vi "Lab 5.vi"() -> ()   [LabVIEW 2025]
uses:
  Control ENUM.ctl
  Lab 3/Control og.ctl
  Lab 3/Control Runners.ctl
  Lab 3/Control Raw.ctl
  <vilib>/Analysis/baseanly.llb/Mean (DBL).vi
  <vilib>/Instr/_visa.llb/VISA Configure Serial Port (Instr).vi
  <vilib>/Analysis/NI_AALBase.lvlib
panel:
  in  "Enter your name":string
  in  "Play":bool
  in  "Button":bool
  out "Waveform Chart":i32(graph)
  out "XY Graph 2":cluster{i32[], i32[]}(graph)
  out "return count":u32
  out "error out 2":errorcluster
  in  "stop":bool
  out "read buffer":string
  out "Cursor BPM":dbl
  in  "Training Data":path
  out "HEART RATE ZONES":string[][](array[string])
  out "BPM":cluster{"Time":timestamp[], "Bpm":i32[]}(graph)
  out "XY Graph":T1(graph)
  in  "Stop":bool
  in  "Save":bool
  in  "New":bool
  out "error out":errorcluster
  in  "error in":errorcluster
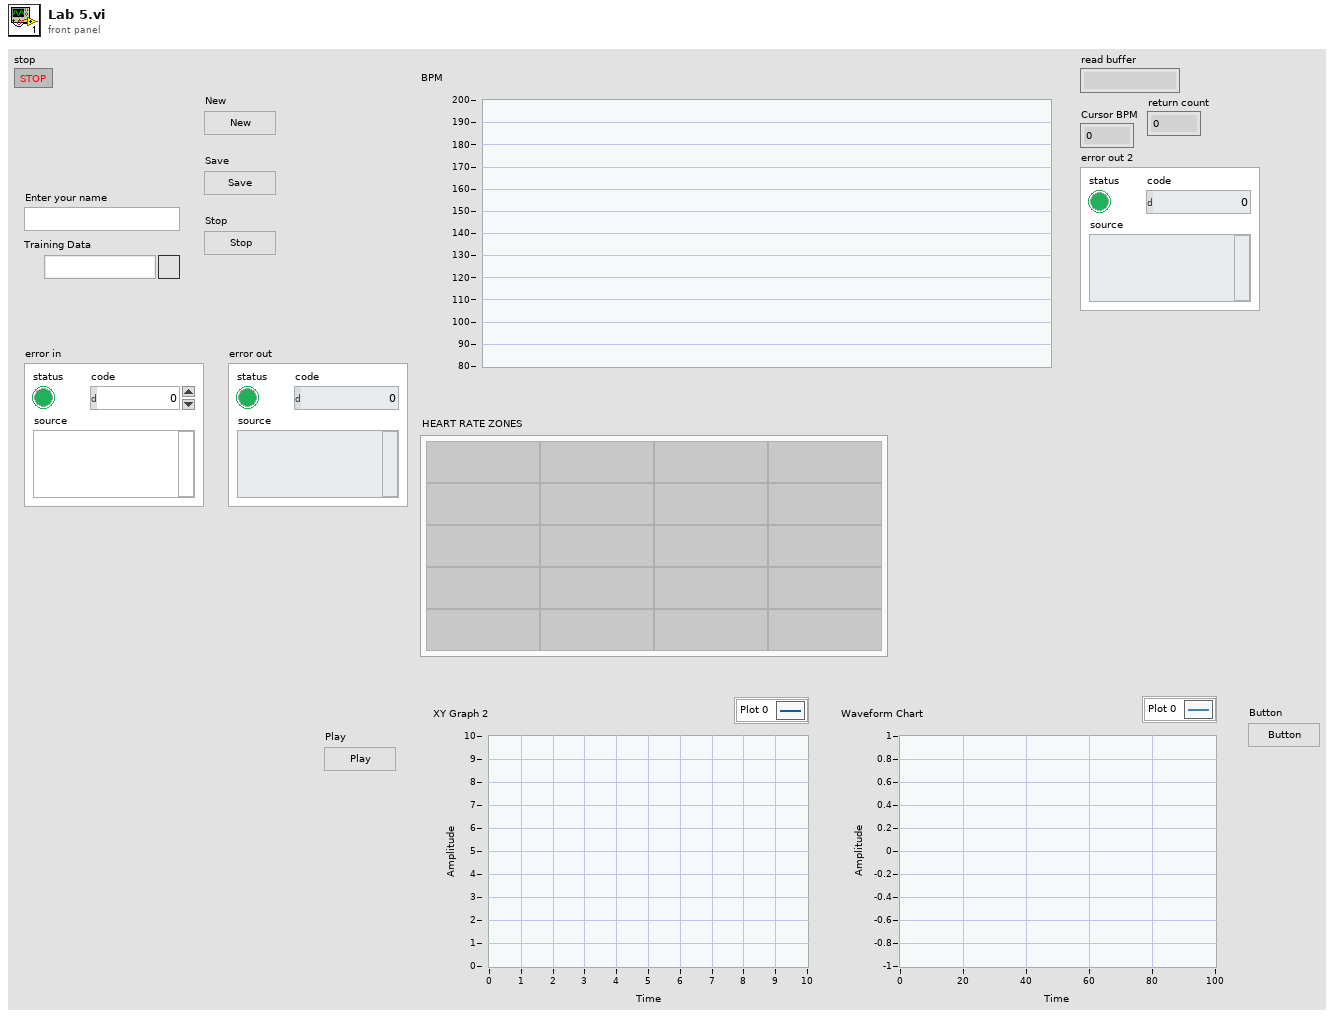
[diagram p1: front panel]
types:
  T1 = cluster{"Total Time in Zone":dbl[], "Heart Rate Zone No":dbl[]}
  T2 = typedef "Control og.ctl" = cluster{"Runner's Data":T3, "HR Max":i32, "Raw Data":T4, "% HR MAX ":dbl[], "HR Zones":string[][], "Heart Rate Zone No":dbl[], "Total Time in Zone":dbl[]}
  T3 = typedef "Control Runners.ctl" = cluster{"Name":string, "Age":i32}
  T4 = typedef "Control Raw.ctl" = cluster{"Time":timestamp[], "Bpm":i32[]}
  T5 = typedef "Control ENUM.ctl" = enum16{"Application Error", "Init", "Idle", "Analyse New Training", "Save", "Error Handling", "Stop", "Play\n"}
  T6 = enum16{"open", "replace", "create", "open or create", "replace or create", "replace or create with confirmation"}
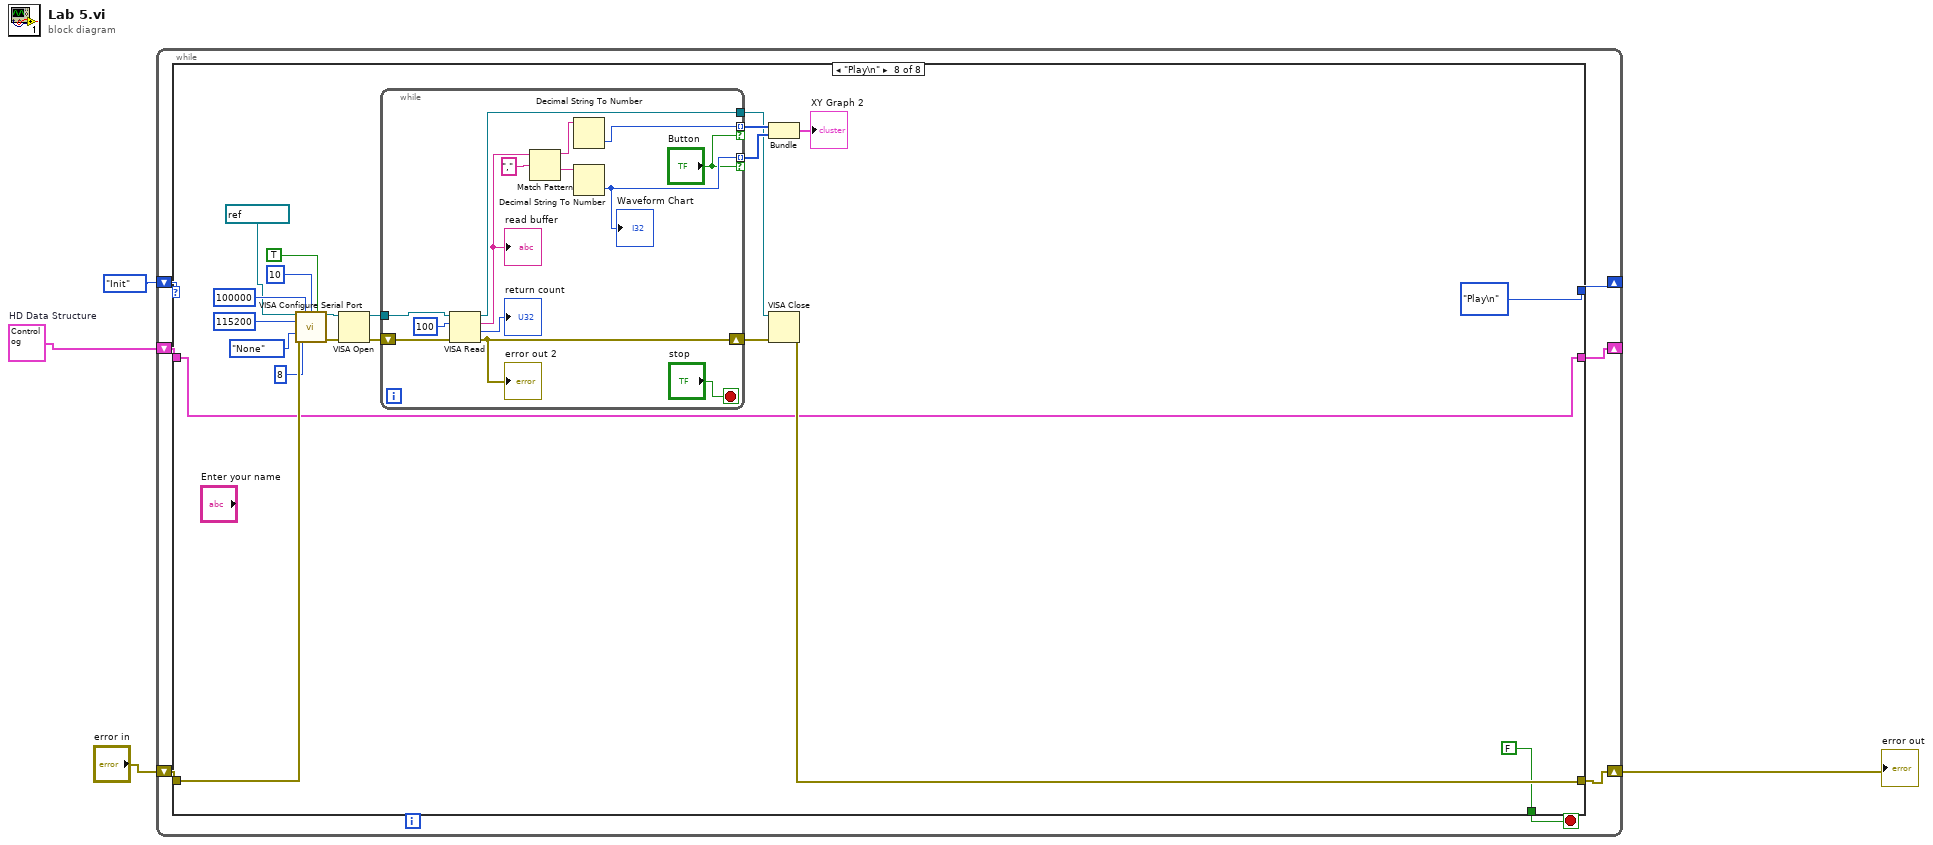
[diagram p0: block diagram]
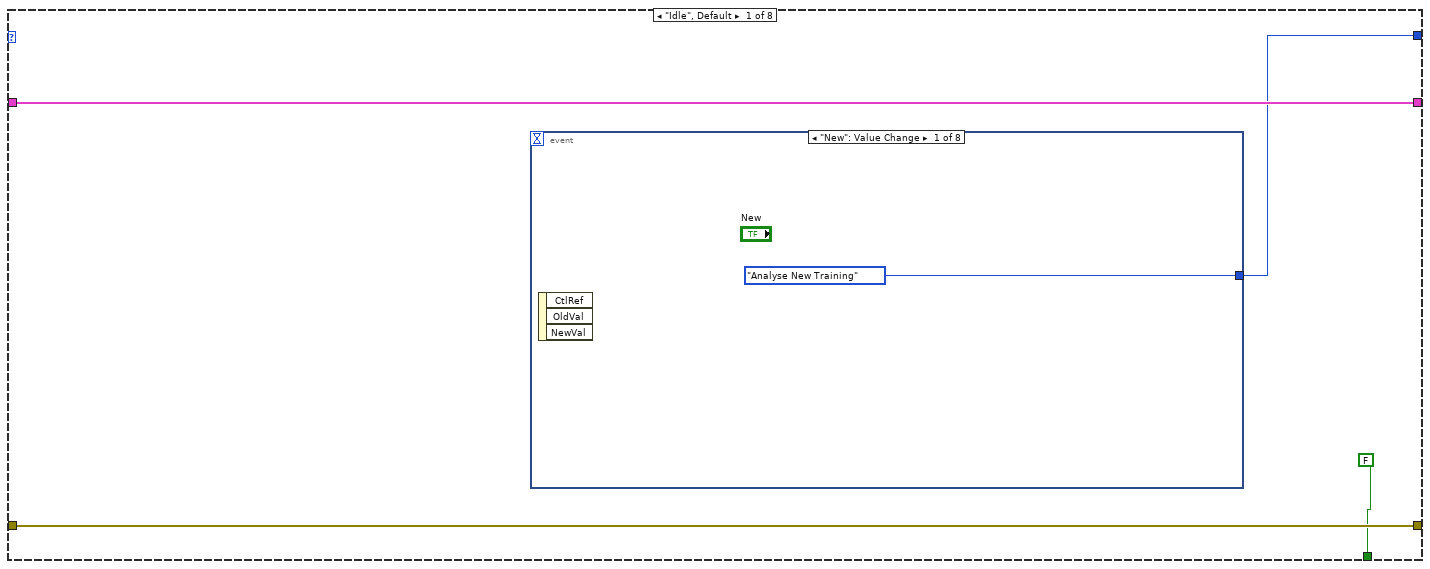
[diagram p2: hidden frame]
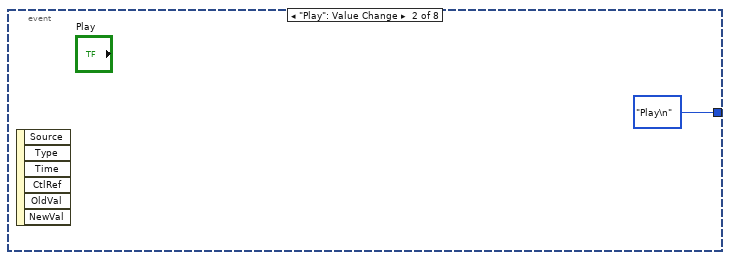
[diagram p3: hidden frame]
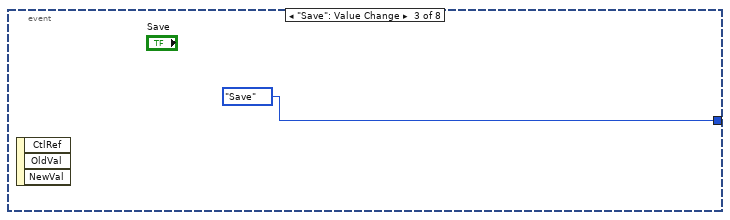
[diagram p4: hidden frame]
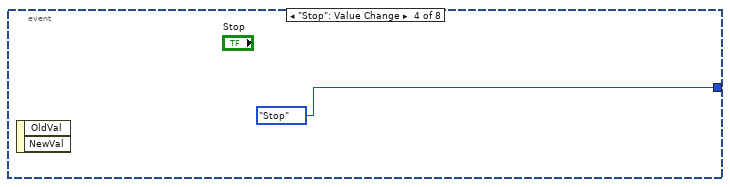
[diagram p5: hidden frame]
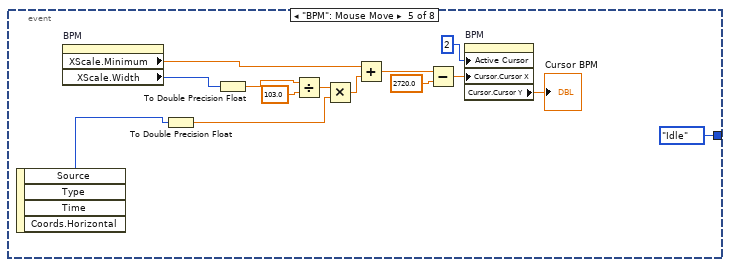
[diagram p6: hidden frame]
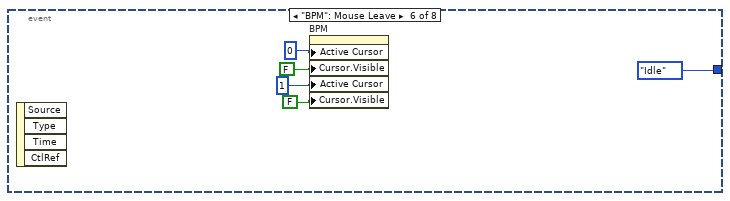
[diagram p7: hidden frame]
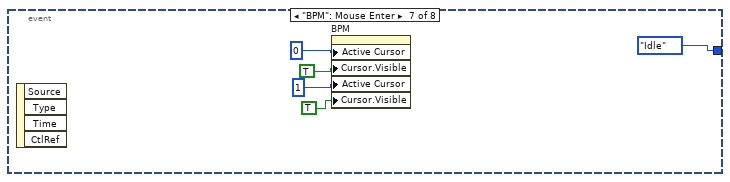
[diagram p8: hidden frame]
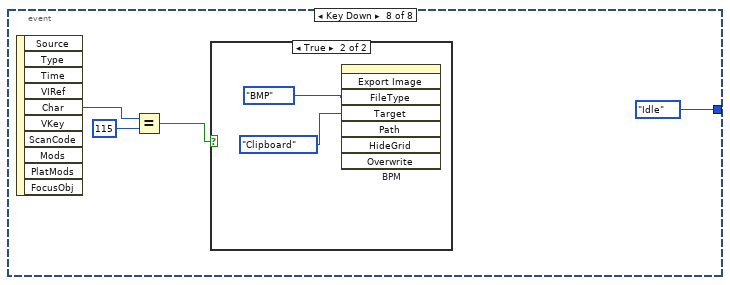
[diagram p9: hidden frame]
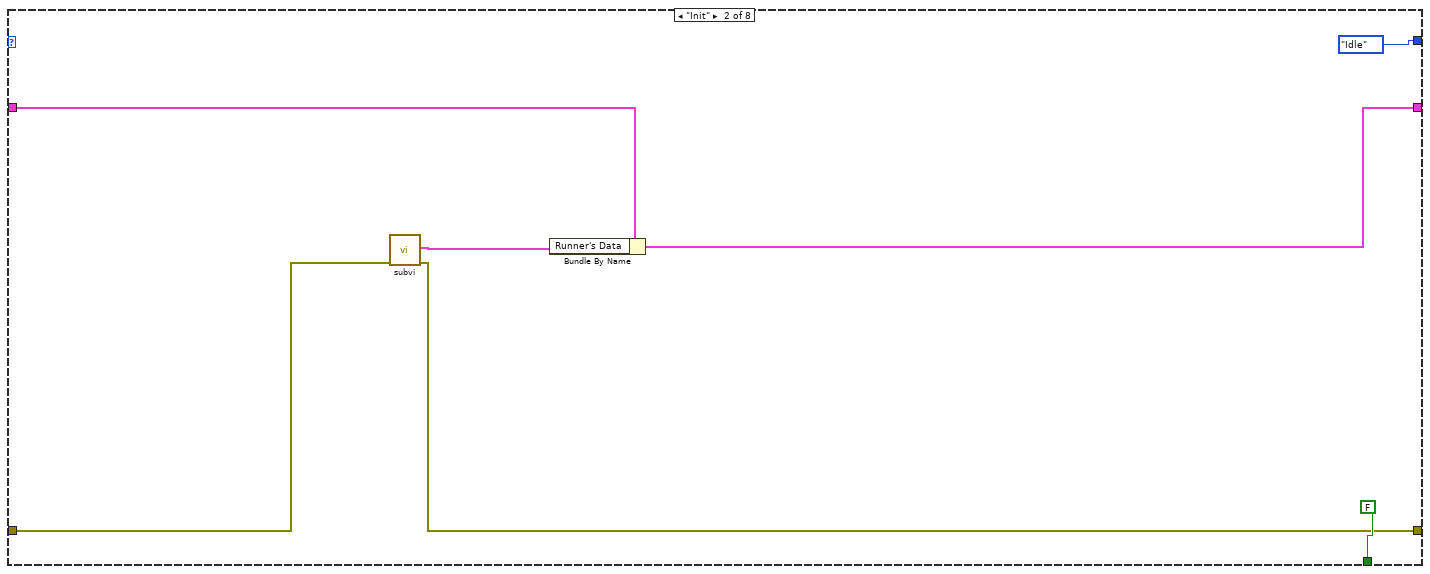
[diagram p11: hidden frame]
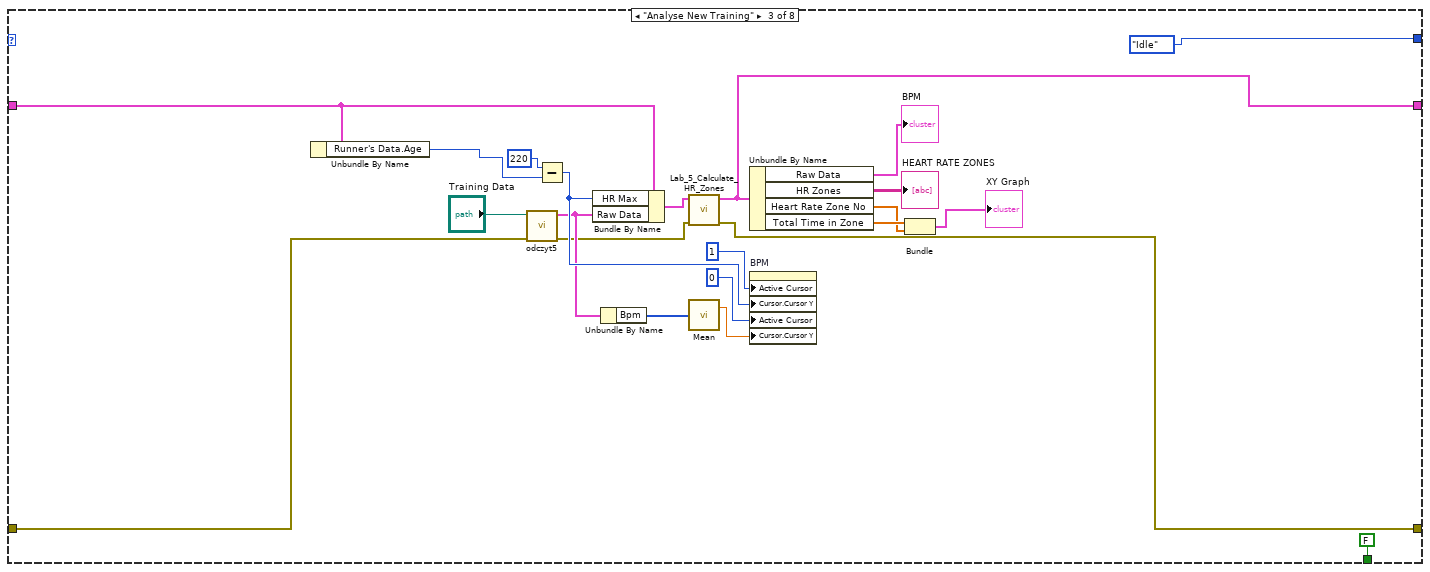
[diagram p12: hidden frame]
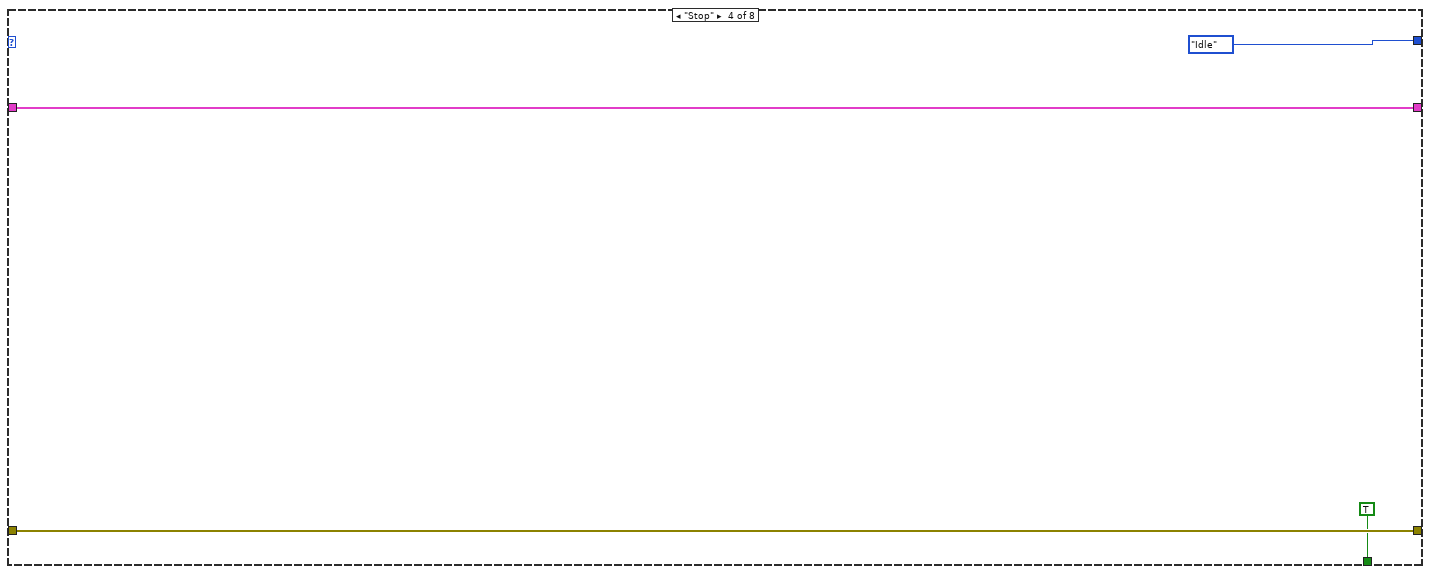
[diagram p13: hidden frame]
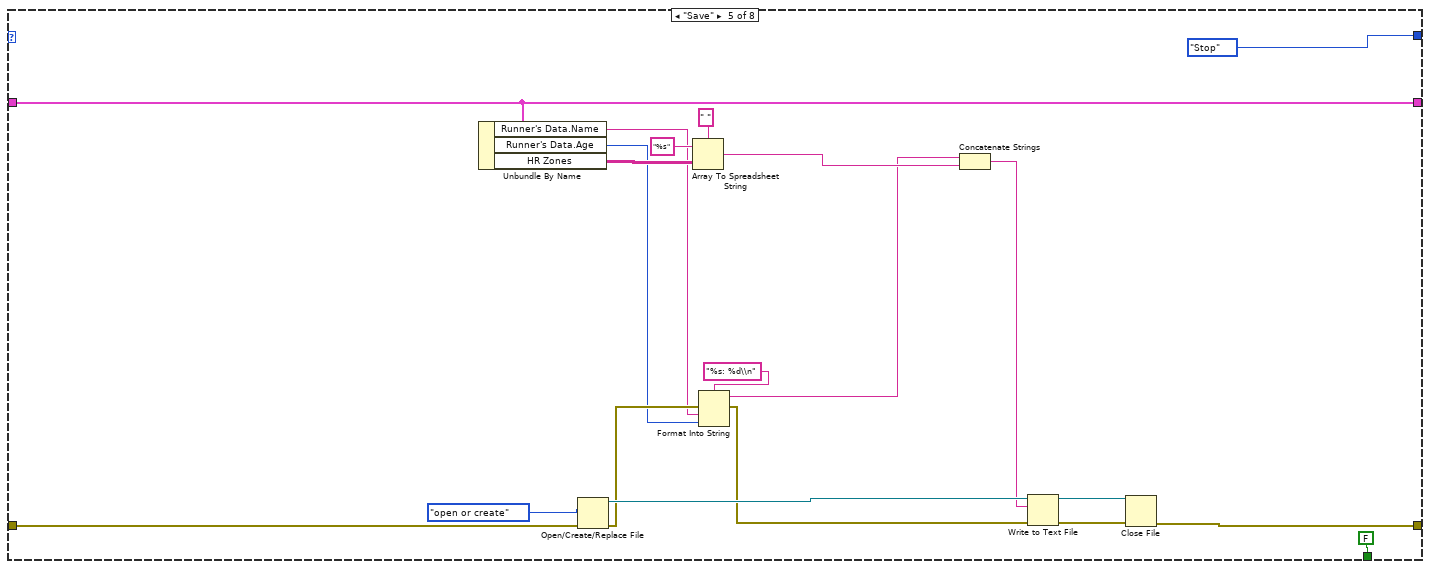
[diagram p14: hidden frame]
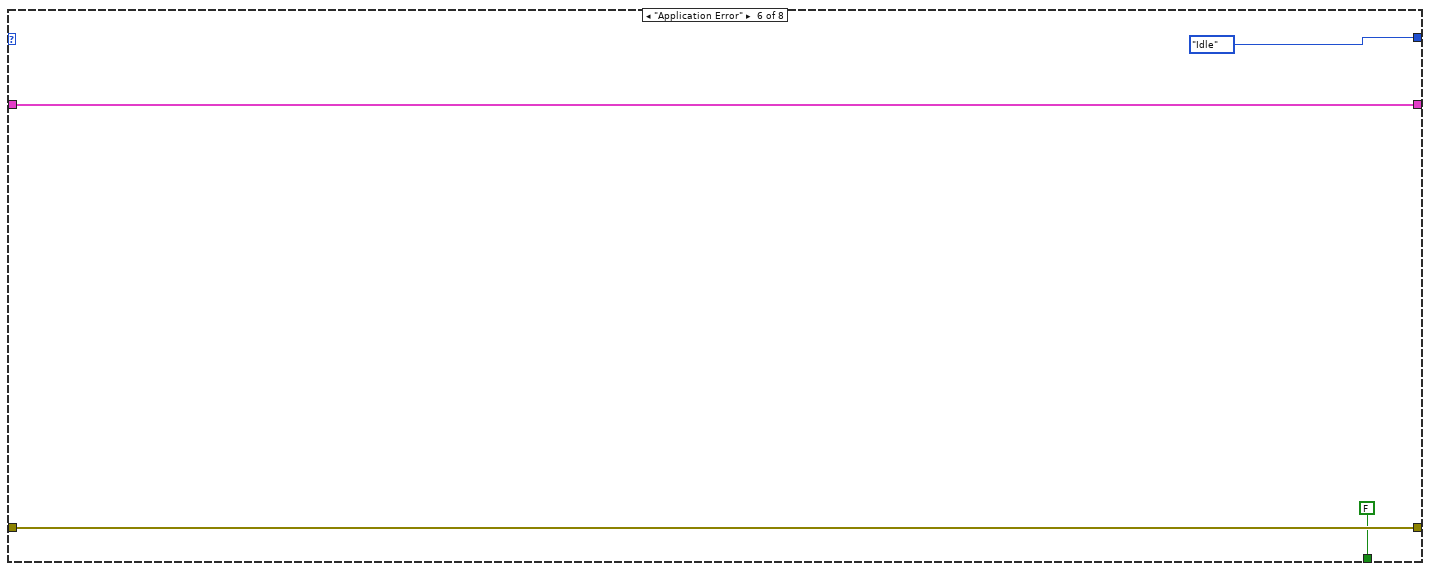
[diagram p15: hidden frame]
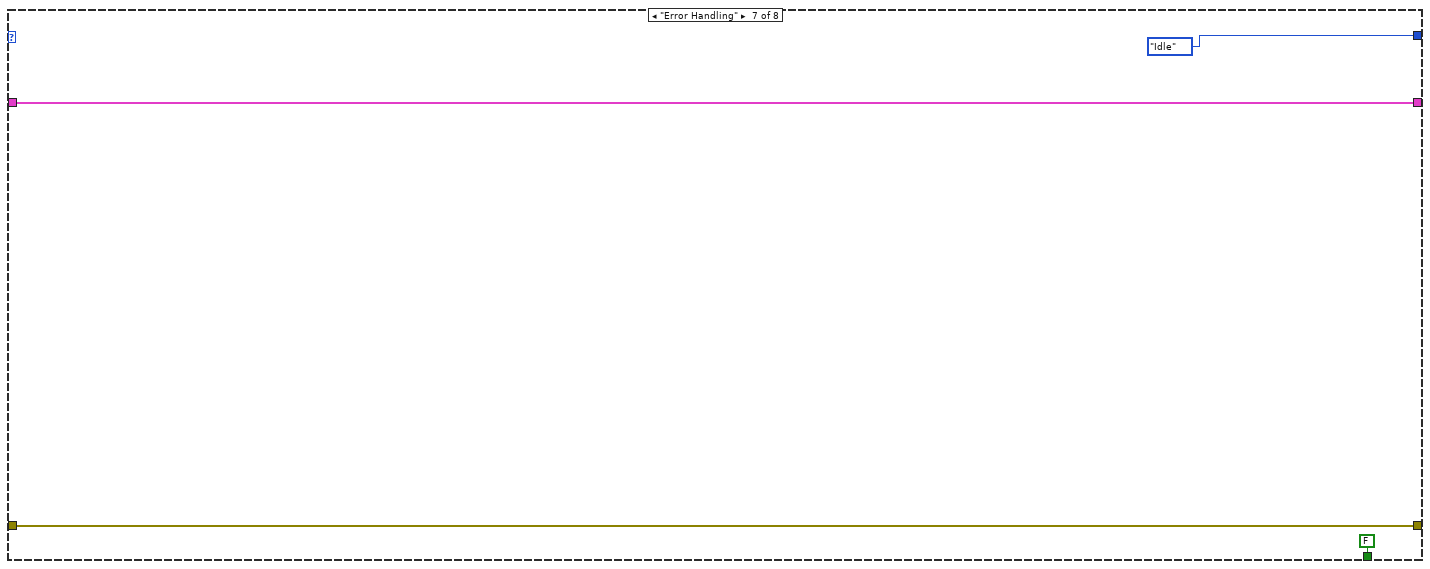
[diagram p16: hidden frame]
diagram:
  w1 = T2 data[18182B]  # HD Data Structure
  n1 = while {
    shift-right: [w11] -> _
    shift-left: w1 -> [w10]
    shift-right: [w8] -> _
    shift-left: Control_ENUM."Init" -> [w9]
    shift-right: [w7] -> w2
    shift-left: "error in" -> [w6]
    stop <- w5 stop-if-true
    n2 = case shown="\"Play\\n\"" w9 {
      tunnel: [w15 w50 w59 w81 w96 w106 w108 w113] -> w11
      tunnel: w10 -> [w15 w51 w58 w81 w96 w106 w108 w113]
      tunnel: [w12 Control_ENUM."Idle" Control_ENUM."Idle" Control_ENUM."Idle" Control_ENUM."Stop" Control_ENUM."Idle" Control_ENUM."Idle" Control_ENUM."Play\n"] -> w8
      tunnel: [w14 w53 w65 w80 w100 w105 w110 w117] -> w7
      tunnel: w6 -> [w14 w54 w62 w80 w99 w105 w110 w118]
      tunnel: [FALSE FALSE FALSE TRUE FALSE FALSE FALSE FALSE] -> w5
      frame "Idle", Default {
        n3 = event shown="[0] \"New\": Value Change" {
          selector: _ -> [_ _ _ _ _ _ _ _]
          dyn-events: _ -> [_ _ _ _ _ _ _ _]
          timeout: _ -> [_ _ _ _ _ _ _ _]
          tunnel: [Control_ENUM."Analyse New Training" Control_ENUM."Play\n" Control_ENUM."Save" Control_ENUM."Stop" Control_ENUM."Idle" Control_ENUM."Idle" Control_ENUM."Idle" Control_ENUM."Idle"] -> w12
          event "New": Value Change {
            n4 = event-data() -> ()  [unwired: 1 in, 3 out]
          }
          event "Play": Value Change {
            n5 = event-data() -> ()  [unwired: 1 in, 6 out]
          }
          event "Save": Value Change {
            n6 = event-data() -> ()  [unwired: 1 in, 3 out]
          }
          event "Stop": Value Change {
            n7 = event-data() -> ()  [unwired: 1 in, 2 out]
          }
          event "BPM": Mouse Move {
            n8 = event-data() -> ("Coords.Horizontal"=w21:i32)  [unwired: 1 in, 3 out]
            n9 = property on="BPM" class="XYGraph (strict)"() -> ("XScale.Minimum"=w29:dbl, "XScale.Width"=w23:u32)  [unwired: 2 in, 2 out]
            n10 = To Double Precision Float(number=w21) -> (double precision float=w20:dbl)
            n11 = To Double Precision Float(number=w23) -> (double precision float=w22:dbl)
            n12 = Divide(x=w22, y=103.0) -> (x/y=w31:dbl)
            n13 = Multiply(x=w31, y=w20) -> (x*y=w30:dbl)
            n14 = Add(x=w29, y=w30) -> (x+y=w28:dbl)
            n15 = Subtract(x=w28, y=2720.0) -> (x-y=w26:dbl)
            n16 = property on="BPM" class="XYGraph (strict)"("Active Cursor"=u32 2, "Cursor.Cursor X"=w26) -> ("Cursor.Cursor Y"=→"Cursor BPM":dbl)  [unwired: 2 in, 2 out]
          }
          event "BPM": Mouse Leave {
            n17 = event-data() -> ()  [unwired: 1 in, 4 out]
            n18 = property on="BPM" class="XYGraph (strict)"("Active Cursor"=u32 0, "Cursor.Visible"=FALSE, "Active Cursor"=u32 1, "Cursor.Visible"=FALSE) -> ()  [unwired: 2 in, 2 out]
          }
          event "BPM": Mouse Enter {
            n19 = event-data() -> ()  [unwired: 1 in, 4 out]
            n20 = property on="BPM" class="XYGraph (strict)"("Active Cursor"=u32 0, "Cursor.Visible"=TRUE, "Active Cursor"=u32 1, "Cursor.Visible"=TRUE) -> ()  [unwired: 2 in, 2 out]
          }
          event Key Down {
            n21 = event-data() -> ("Char"=w45:i16)  [unwired: 1 in, 9 out]
            n22 = Equal?(x=w45, y=i16 115 ("ScanCode")) -> (x = y?=w46:bool)
            n23 = case shown="True" w46 {
              frame False {
              }
              frame True {
                n24 = invoke on="BPM" class="XYGraph (strict)" method="Export Image"("FileType"=enum32{"BMP", "EPS", "EMF", "PICT"}."BMP" ("File Type"), "Target"=enum32{"File", "Clipboard"}."Clipboard") -> ()  [unwired: 6 in, 8 out]
              }
            }
          }
        }
      }
      frame "Init" {
        n25 = call "subvi.vi"("error in"=w54) -> ("error out"=w53:errorcluster, "Runner's Data Ind"=w52:T3)  [unwired: 9 in]
        n26 = Bundle By Name(cluster=w51, "Runner's Data"=w52) -> (w50:T2)
      }
      frame "Analyse New Training" {
        n27 = Unbundle By Name(w58) -> ("Runner's Data.Age"=w57:i32)
        n28 = call "odczyt5.vi"("error in"=w62, "Path"="Training Data") -> ("error out"=w61:errorcluster, "Raw Data"=w63:T4)  [unwired: 8 in]
        n29 = Subtract(x=220, y=w57) -> (x-y=w75:i32)
        n30 = Bundle By Name(cluster=w58, "HR Max"=w75, "Raw Data"=w63) -> (w66:T2)
        n31 = Unbundle By Name(w63) -> ("Bpm"=w76:i32[])
        n32 = call "Lab_5_Calculate_HR_Zones.vi"("error in"=w61, "HD Data Structure"=w66) -> ("error out"=w65:errorcluster, "HD Data Structure"=w59:T2)  [unwired: 8 in]
        n33 = call-poly <vilib>:"Mean.vi"("X"=w76) -> ("mean"=w77:dbl)  [unwired: 1 out]
        n34 = Unbundle By Name(w59) -> ("Raw Data"=→"BPM":T4, "HR Zones"=→"HEART RATE ZONES":string[][], "Heart Rate Zone No"=w72:dbl[], "Total Time in Zone"=w73:dbl[])
        n35 = property on="BPM" class="XYGraph (strict)"("Active Cursor"=u32 1, "Cursor.Cursor Y"=w75, "Active Cursor"=u32 0, "Cursor.Cursor Y"=w77) -> ()  [unwired: 2 in, 2 out]
        n36 = Bundle("Total Time in Zone"=w73, "Heart Rate Zone No"=w72) -> (→"XY Graph":T1)  [unwired: 1 in]
      }
      frame "Stop" {
      }
      frame "Save" {
        n37 = Unbundle By Name(w96) -> ("Runner's Data.Name"=w90:string, "Runner's Data.Age"=w91:i32, "HR Zones"=w95:string[][])
        n38 = Open/Create/Replace File(error in=w99, operation (0:open)=T6."open or create") -> (refnum out=w102:refnum<file>, error out=w92:errorcluster)  [unwired: 4 in, 1 out]
        n39 = Array To Spreadsheet String(delimiter (Tab)=" ", array=w95, 3:"%s" ("format string")) -> (spreadsheet string=w93:string)
        n40 = Format Into String(format string="%s: %d\\n", error in=w92, w90, w91) -> (resulting string=w88:string, error out=w85:errorcluster)  [unwired: 1 in]
        n41 = Concatenate Strings(w88, w93) -> (w87:string)
        n42 = Write to Text File(file (use dialog)=w102, text=w87, error in=w85) -> (refnum out=w101:refnum<file>, error out=w84:errorcluster)  [unwired: 1 in, 1 out]
        n43 = Close File(refnum=w101, error in=w84) -> (error out=w100:errorcluster)  [unwired: 1 out]
      }
      frame "Application Error" {
      }
      frame "Error Handling" {
      }
      frame "Play\n" {
        n44 = call-poly "VISA Configure Serial Port"("VISA resource name"=refnum<visa-resource-name> "COM3", "timeout (10sec)"=u32 100000, "termination char\n(0xA = '\\n' = LF)"=u8 10 ("termination char\n(0xA = '\\n' = LF)"), "Enable Termination\nChar (T)"=TRUE ("Enable Termination\nChar (T)"), "baud rate (9600)"=u32 115200, "data bits (8)"=u16 8, "parity (0:none)"=enum16{"None", "Odd", "Even", "Mark", "Space"}."None", "error in (no error)"=w118) -> ("VISA resource name out"=w124:refnum<visa-resource-name>, "error out"=w123:errorcluster)  [unwired: 6 in]
        n45 = VISA Open(error in (no error)=w123, VISA resource name=w124) -> (VISA resource name=w125:refnum<visa-resource-name>, error out=w128:errorcluster)  [unwired: 3 in]
        n46 = while {
          tunnel: w125 -> [w144]
          tunnel: [w143] -> w127
          shift-right: [w140] -> w126
          shift-left: w128 -> [w142]
          tunnel: [w134] -> w130 mode=indexing if="Button"
          tunnel: [w133] -> w131 mode=indexing if="Button"
          stop <- "stop" stop-if-true
          n47 = VISA Read(VISA resource name=w144, byte count=u32 100, error in (no error)=w142) -> (VISA resource name out=w143:refnum<visa-resource-name>, read buffer=w138:string, return count=→"return count":u32, error out=w140:errorcluster)
          "read buffer" <- w138
          "error out 2" <- w140
          n48 = Match Pattern(string=w138, regular expression=",") -> (before substring=w136:string, after substring=w135:string)  [unwired: 1 in, 2 out]
          n49 = Decimal String To Number(string=w136) -> (number=w133:i32)  [unwired: 2 in, 1 out]
          n50 = Decimal String To Number(string=w135) -> (number=w134:i32)  [unwired: 2 in, 1 out]
          "Waveform Chart" <- w134
        }
        n51 = Bundle(w131, w130) -> (→"XY Graph 2":cluster{i32[], i32[]})  [unwired: 1 in]
        n52 = VISA Close(VISA resource name=w127, error in (no error)=w126) -> (error out=w117:errorcluster)
      }
    }
  }
  "error out" <- w2
